vi "Get Tree Data for Affected Item.vi"(7 "Action":T2, 10 "User VI Ref":refnum<vi>, 11 "Affected Items":T3) -> (2 "Use Dialog?":bool, 3 "Elements Array":T1[](array[typedef]))   [LabVIEW 2023]
doc: "Given one of the affected items, return the associated cluster type of that item.\n\nIf action is Rearrange or Delete, this will be an array of strings of the bundle or unbundle by name terminals."
uses:
  top/BundleMagic.ctl
  controls/action enum.ctl
  cluster/Cluster Element Description.ctl
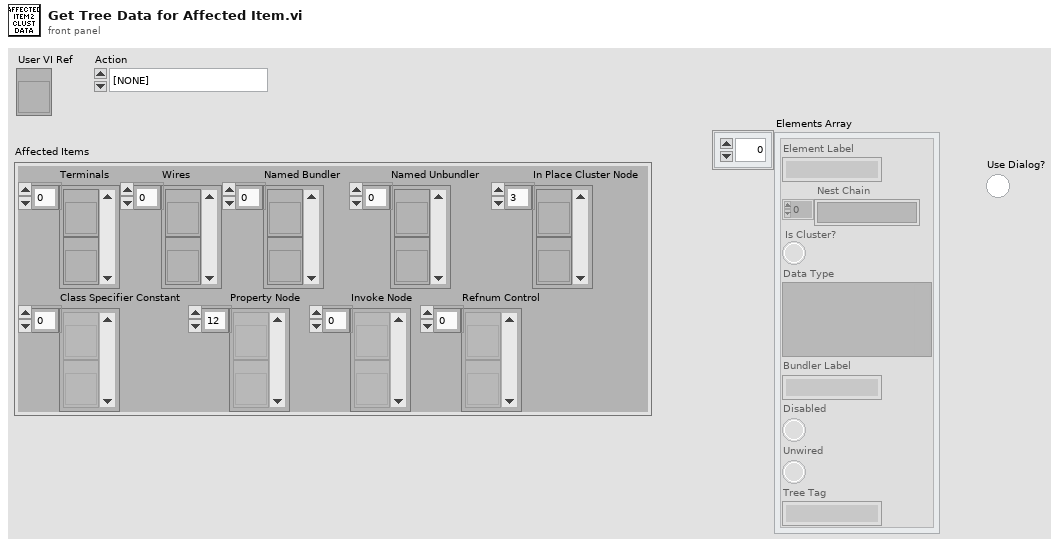
[diagram p1: front panel]
types:
  T1 = typedef "Cluster Element Description.ctl" = cluster{"Element Label":string, "Nest Chain":string[], "Is Cluster?":bool, "Data Type":variant, "Bundler Label":string, "Disabled":bool, "Unwired":bool, "Tree Tag":string}
  T2 = typedef "action enum.ctl" = enum16{"[NONE]", "Wire Bundle", "Wire Unbundle", "Terminal Unbundle", "Terminal Bundle", "Bundler Move Up", "Bundler Move Down", "Bundler Insert", "Bundler Remove", "Bundler Remove Unwired", "Bundler Rearrange", "In Place Insert", "In Place Remove", "In Place Remove Unwired", "In Place Rearrange", "Wire Properties", "Wire Method", "Terminal Properties", "Terminal Method", "Property Move Up", "Property Move Down", "Properties Insert", "Properties Remove", "Properties Remove Unwired", "Properties Rearrange", "Method Change", "Class For Constant", "Class For Control", "Class For Node", "Class Name to Clipboard"}
  T3 = typedef "BundleMagic.ctl" = cluster{"Terminals":refnum<vi>[], "Wires":refnum<vi>[], "Named Bundler":refnum<vi>[], "Named Unbundler":refnum<vi>[], "In Place Cluster Node":refnum<vi>[], "Class Specifier Constant":refnum<vi>[], "Property Node":refnum<vi>[], "Invoke Node":refnum<vi>[], "Refnum Control":refnum<vi>[]}
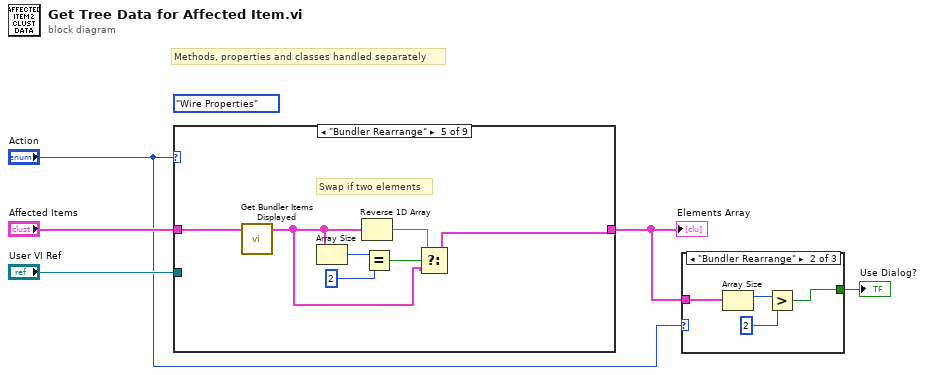
[diagram p0: block diagram]
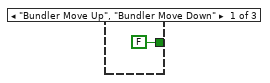
[diagram p2: hidden frame]
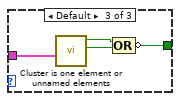
[diagram p3: hidden frame]
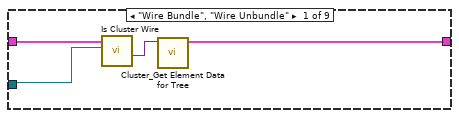
[diagram p4: hidden frame]
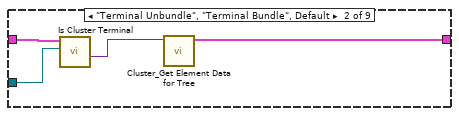
[diagram p5: hidden frame]
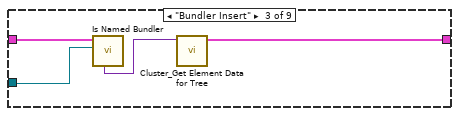
[diagram p6: hidden frame]
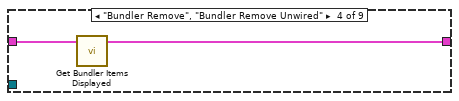
[diagram p7: hidden frame]
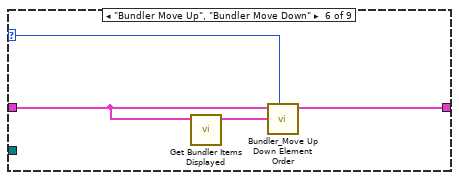
[diagram p8: hidden frame]
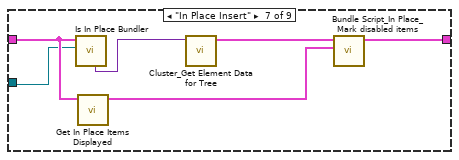
[diagram p9: hidden frame]
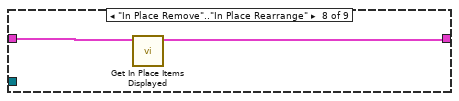
[diagram p10: hidden frame]
diagram:
  (unwired) action_enum."Wire Properties" ("Action")
  # "Methods, properties and classes handled separately"
  n1 = case shown="\"Bundler Rearrange\"" "Action" {
    selector: "Action" -> [_ _ _ _ _ w30 _ _ _]
    tunnel: "Affected Items" -> [w9 w13 w17 w19 w26 w27 w35 w38 _]
    tunnel: "User VI Ref" -> [w8 w12 w16 _ _ _ w33 _ _]
    tunnel: [w6 w10 w14 w18 w20 w29 w34 w37 _] -> w2
    frame "Wire Bundle", "Wire Unbundle" {
      n2 = call "Is Cluster Wire.vi"("User VI Ref"=w8, "Affected Items"=w9) -> ("Data Type"=w7:variant)  [unwired: 6 in, 3 out]
      n3 = call "Cluster_Get Element Data for Tree.vi"("Data Type"=w7) -> ("Cluster Element Data Aray"=w6:T1[])  [unwired: 10 in]
    }
    frame "Terminal Unbundle", "Terminal Bundle", Default {
      n4 = call "Is Cluster Terminal.vi"("User VI Ref"=w12, "Affected Items"=w13) -> ("Data Type"=w11:variant)  [unwired: 7 in, 2 out]
      n5 = call "Cluster_Get Element Data for Tree.vi"("Data Type"=w11) -> ("Cluster Element Data Aray"=w10:T1[])  [unwired: 10 in]
    }
    frame "Bundler Insert" {
      n6 = call "Is Named Bundler.vi"("User VI Ref"=w16, "Affected Items"=w17) -> ("Data Type"=w15:variant)  [unwired: 3 in, 6 out]
      n7 = call "Cluster_Get Element Data for Tree.vi"("Data Type"=w15) -> ("Cluster Element Data Aray"=w14:T1[])  [unwired: 10 in]
    }
    frame "Bundler Remove", "Bundler Remove Unwired" {
      n8 = call "Get Bundler Items Displayed.vi"("Affected Items"=w19) -> ("Displayed Items"=w18:T1[])  [unwired: 10 in]
    }
    frame "Bundler Rearrange" {
      # "Swap if two elements"
      n9 = call "Get Bundler Items Displayed.vi"("Affected Items"=w26) -> ("Displayed Items"=w21:T1[])  [unwired: 10 in]
      n10 = Array Size(array=w21) -> (size(s)=w25:i32)
      n11 = Reverse 1D Array(array=w21) -> (reversed array=w22:T1[])
      n12 = Equal?(x=w25, y=2) -> (x = y?=w23:bool)
      n13 = Select(t=w22, s=w23, f=w21) -> (s? t:f=w20:T1[])
    }
    frame "Bundler Move Up", "Bundler Move Down" {
      n14 = call "Get Bundler Items Displayed.vi"("Affected Items"=w27) -> ("Displayed Items"=w28:T1[])  [unwired: 10 in]
      n15 = call "Bundler_Move Up Down Element Order.vi"("Action"=w30, "Cluster Elements In"=w28, "Affected Items"=w27) -> ("Cluster Elements Out"=w29:T1[])  [unwired: 8 in]
    }
    frame "In Place Insert" {
      n16 = call "Is In Place Bundler.vi"("User VI Ref"=w33, "Affected Items"=w35) -> ("Data Type"=w32:variant)  [unwired: 6 in, 3 out]
      n17 = call "Get In Place Items Displayed.vi"("Affected Items"=w35) -> ("Displayed Items"=w36:T1[])  [unwired: 10 in]
      n18 = call "Cluster_Get Element Data for Tree.vi"("Data Type"=w32) -> ("Cluster Element Data Aray"=w31:T1[])  [unwired: 10 in]
      n19 = call "Bundle Script_In Place_Mark disabled items.vi"("Displayed Items"=w36, "Cluster Items"=w31) -> ("Dialog Items"=w34:T1[])  [unwired: 9 in]
    }
    frame "In Place Remove".."In Place Rearrange" {
      n20 = call "Get In Place Items Displayed.vi"("Affected Items"=w38) -> ("Displayed Items"=w37:T1[])  [unwired: 10 in]
    }
    frame "[NONE]" {
    }
  }
  "Elements Array" <- w2
  n21 = case shown="\"Bundler Rearrange\"" "Action" {
    tunnel: [FALSE w40 w45] -> w3
    tunnel: w2 -> [_ w43 w44]
    frame "Bundler Move Up", "Bundler Move Down" {
    }
    frame "Bundler Rearrange" {
      n22 = Array Size(array=w43) -> (size(s)=w42:i32)
      n23 = Greater?(x=w42, y=2) -> (0:w40:bool)
    }
    frame Default {
      n24 = call "Cluster is one element or unnamed elements.vi"("Cluster Elements Array"=w44) -> ("All Unnamed?"=w46:bool, "One Element?"=w47:bool)  [unwired: 8 in, 1 out]
      n25 = Compound Arithmetic op=OR(w47, w46) -> (invert w45:bool)
    }
  }
  "Use Dialog?" <- w3
